vi "Results_Get_ReadFull.vi"(8 "error in (no error)":errorcluster, 11 "appended array":dbl[](array[numeric])) -> (0 "error out":errorcluster, 1 "Fault Data":T1[](array[typedef]), 2 "Motion I/O":T3[](array[typedef]), 3 "Feedback":T2[](array[typedef]))   [LabVIEW 2017, in "WordManipulationLibrary.lvlib"]
uses:
  WordManipulationLibrary.lvlib
  Results_MotionIO.ctl
  Results_Trajectory.ctl
  Results_Faults.ctl
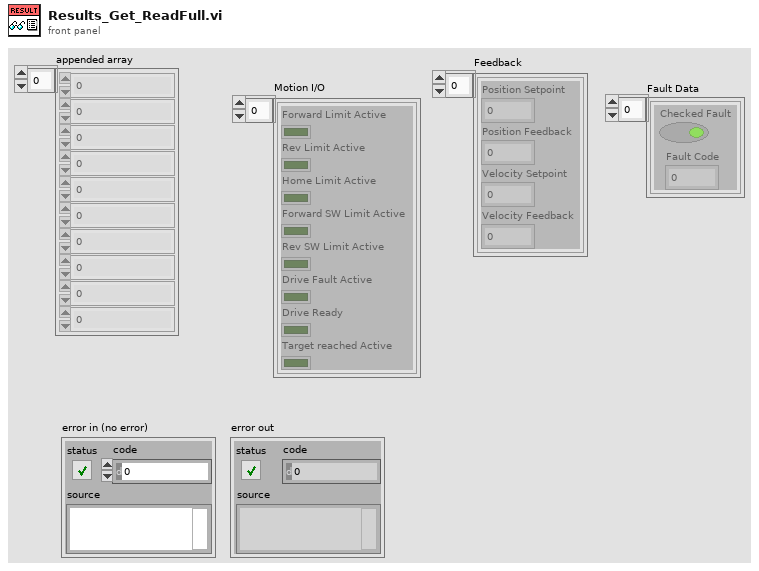
[diagram p1: front panel]
types:
  T1 = typedef "WordManipulationLibrary.lvlib/Results_Faults.ctl" = cluster{"Checked Fault":bool, "Fault Code":i32}
  T2 = typedef "WordManipulationLibrary.lvlib/Results_Trajectory.ctl" = cluster{"Position Setpoint":dbl, "Position Feedback":dbl, "Velocity Setpoint":dbl, "Velocity Feedback":dbl}
  T3 = typedef "WordManipulationLibrary.lvlib/Results_MotionIO.ctl" = cluster{"Forward Limit Active":bool, "Rev Limit Active":bool, "Home Limit Active":bool, "Forward SW Limit Active":bool, "Rev SW Limit Active":bool, "Drive Fault Active":bool, "Drive Ready":bool, "Target reached Active":bool}
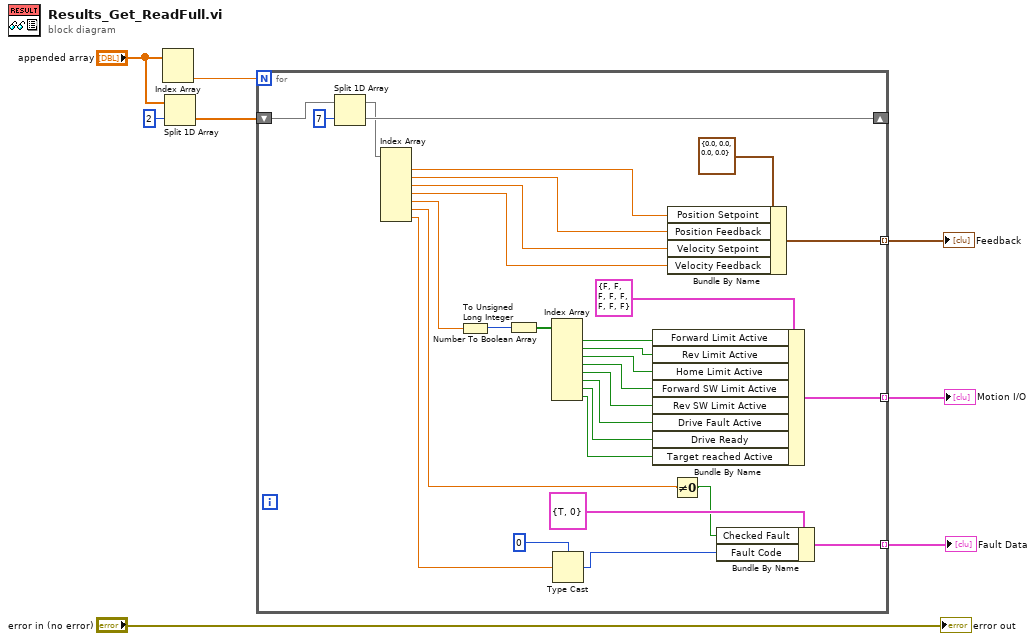
[diagram p0: block diagram]
diagram:
  n1 = Index Array(array="appended array") -> (element #2=w2:dbl)  [unwired: 2 in, 1 out]
  n2 = Split 1D Array(array="appended array", index=2) -> (second subarray=w5:dbl[])  [unwired: 1 out]
  n3 = for {
    N: w2 -> [_]
    tunnel: [w37] -> w3 mode=indexing
    tunnel: [w25] -> w4 mode=indexing
    shift-right: [w22] -> _
    shift-left: w5 -> [w24]
    tunnel: [w13] -> w1 mode=indexing
    n4 = Split 1D Array(array=w24, index=7) -> (first subarray=w21:dbl[], second subarray=w22:dbl[])
    n5 = Index Array(array=w21) -> (element #1=w20:dbl, element #2=w19:dbl, element #3=w18:dbl, element #4=w9:dbl, element #5=w12:dbl, element #6=w10:dbl, element #7=w11:dbl)  [unwired: 7 in]
    n6 = To Unsigned Long Integer(number=w12) -> (unsigned 32bit integer=w36:u32)
    n7 = Number To Boolean Array(number=w36) -> (Boolean array=w34:bool[])
    n8 = Index Array(array=w34) -> (element #1=w33:bool, element #2=w32:bool, element #3=w31:bool, element #4=w30:bool, element #5=w29:bool, element #6=w28:bool, element #7=w27:bool, element #8=w26:bool)  [unwired: 8 in]
    n9 = Type Cast(type=0 ("Fault Code"), x=w11) -> (*(type *) &x=w14:i32)
    n10 = Bundle By Name(cluster=T3 {"Forward Limit Active"=FALSE, "Rev Limit Active"=FALSE, "Home Limit Active"=FALSE, "Forward SW Limit Active"=FALSE, "Rev SW Limit Active"=FALSE, "Drive Fault Active"=FALSE, "Drive Ready"=FALSE, "Target reached Active"=FALSE} ("MotionIO"), "Forward Limit Active"=w33, "Rev Limit Active"=w32, "Home Limit Active"=w31, "Forward SW Limit Active"=w30, "Rev SW Limit Active"=w29, "Drive Fault Active"=w28, "Drive Ready"=w27, "Target reached Active"=w26) -> (w25:T3)
    n11 = Bundle By Name(cluster=T2 {"Position Setpoint"=0.0, "Position Feedback"=0.0, "Velocity Setpoint"=0.0, "Velocity Feedback"=0.0}, "Position Setpoint"=w20, "Position Feedback"=w19, "Velocity Setpoint"=w18, "Velocity Feedback"=w9) -> (w37:T2)
    n12 = Not Equal To 0?(x=w10) -> (x != 0?=w16:bool)
    n13 = Bundle By Name(cluster=T1 {"Checked Fault"=TRUE, "Fault Code"=0}, "Checked Fault"=w16, "Fault Code"=w14) -> (w13:T1)
  }
  "Motion I/O" <- w4
  "Feedback" <- w3
  "Fault Data" <- w1
  "error out" <- "error in (no error)"
